vi "Call Vaa3D.vi"(8 "error in (no error)":errorcluster, 9 "spacing_between_points":dbl, 10 "Call_Vaa3D":bool, 11 "Z-stack folder path":path) -> (0 "error out":errorcluster)   [LabVIEW 2020]
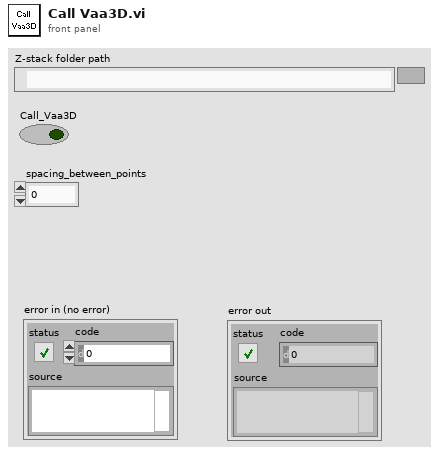
[diagram p1: front panel]
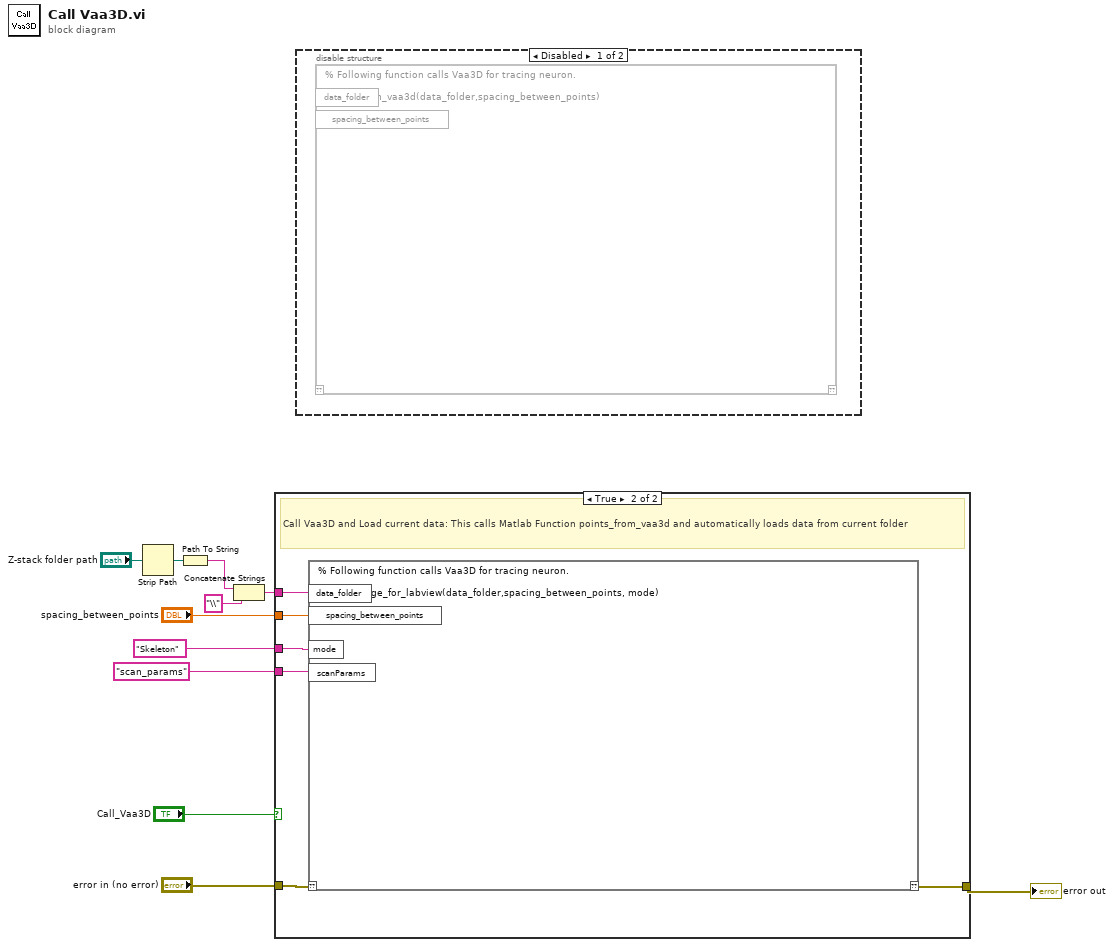
[diagram p0: block diagram]
diagram:
  n1 = Strip Path(path="Z-stack folder path") -> (stripped path=w5:path)  [unwired: 1 out]
  n2 = Path To String(path=w5) -> (string=w6:string)
  n3 = Concatenate Strings(w6, "\\" ("string")) -> (w4:string)
  n4 = case shown="True" "Call_Vaa3D" {
    tunnel: "spacing_between_points" -> [_ w18]
    tunnel: w4 -> [_ w15]
    tunnel: [w12 w17] -> w8
    tunnel: "error in (no error)" -> [w12 w16]
    tunnel: "Skeleton" ("String") -> [_ w14]
    tunnel: "scan_params" ("String") -> [_ w13]
    frame False {
    }
    frame True {
      # "Call Vaa3D and Load current data: This calls Matlab Function points_from_vaa3d and automatically loads data from current folder"
      n5 = script code="% Following function calls Vaa3D for tracing neuron.\n\nvaa3d_bridge_for_labview(data_folder,spacing_between_points, mode)"("??"=w16, "spacing_between_points"=w18, "data_folder"=w15, "mode"=w14, "scanParams"=w13) -> ("??"=w17:errorcluster)
    }
  }
  "error out" <- w8
  n6 = disable-structure shown="Disabled" {
    frame Disabled {
      n7 = script code="% Following function calls Vaa3D for tracing neuron.\n\npoints_from_vaa3d(data_folder,spacing_between_points)"() -> ()  [unwired: 3 in, 1 out]
    }
    frame Enabled {
    }
  }
